vi "VHistory - History Info.vi"(7 "VC Handle":T2=-1, 8 "error in":errorcluster, 11 "name_spec":string) -> (0 "error out":errorcluster, 1 "valid history":bool, 2 "history info":T1 {"oldest timestamp" format="%<%H:%M:%S%2u\n%d/%m/%Y>T"; "NewVals mode"."last read time" format="%<%H:%M:%S%2u\n%d/%m/%Y>T"; "newest timestamp" format="%<%H:%M:%S%2u\n%d/%m/%Y>T"}, 3 "dup name_spec":string, 4 "more data":cluster{"store Writer IDs":bool})   [LabVIEW 2021]
doc: "This VI returns information about a variable history. The VI does not return an error if the specified variable does not have a history attached. Refer to the VI help for more details.\n\n<b>VC Handle</b> specifies the handle of the variable context. To operate on a global variable, pass -1 to this input. This input is ignored if the <b>name_spec</b> control refers to a variable by an alias.\n\n<b>name_spec</b> is the name specifier of the desired variable. Usually, it is merely a variable name; however, its generic format is '[name][=alias]', where either 'name' or '=alias' can be omitted but not both.\n\n<b>history info</b> indicator returns information about both the configuration and state of the history.\n\n<b>valid history</b> indicator returns TRUE if the variable has a history attached.\n\n<b>more data</b> indicator is a cluster containing only the <b>store Writer IDs</b> member, which indicates whether the history stores writer IDs.\n\n::: CalcExpress Toolkit :::\nCopyright (c) 2000-2026 Konstantin Shifershteyn. All rights reserved."
uses:
  cetypes.llb/VarMan Variable Context Handle.ctl
  cetypes.llb/VarMan History Info.ctl
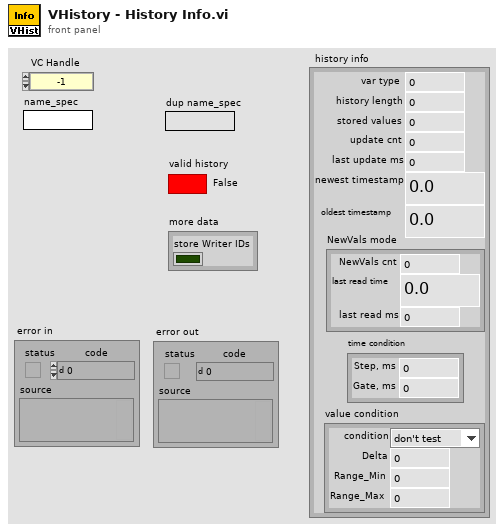
[diagram p1: front panel]
types:
  T1 = typedef "VarMan History Info.ctl" = cluster{"var type":u32, "history length":u32, "stored values":u32, "update cnt":u32, "last update ms":u32, "newest timestamp":dbl, "oldest timestamp":dbl, "NewVals mode":cluster{"NewVals cnt":u32, "last read time":dbl, "last read ms":u32}, "time condition":cluster{"Step, ms":u32, "Gate, ms":u32}, "value condition":cluster{"condition":enum32{"don't test", "changed", "abs deviation", "rel deviation", "out of range", "within range"}, "Delta":dbl, "Range_Min":dbl, "Range_Max":dbl}}
  T2 = typedef "VarMan Variable Context Handle.ctl" = i32
  T3 = enum32{"nop", "create", "destroy", "reset", "get info", "config", "create_wrid"}
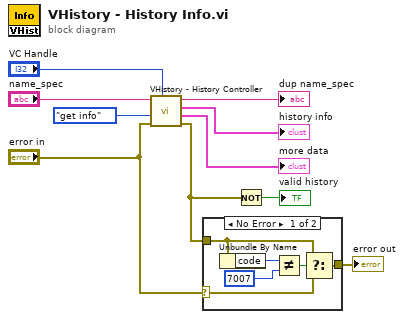
[diagram p0: block diagram]
diagram:
  n1 = call "VHistory - History Controller.vi"("VC Handle"="VC Handle", "error in"="error in", "cmd (nop:default)"=T3."get info", "name_spec"="name_spec") -> ("error out"=w3:errorcluster, "more data"=→"more data":cluster{"store Writer IDs":bool}, "history info"=→"history info":T1, "dup name_spec"=→"dup name_spec":string)  [unwired: 4 in]
  n2 = case shown="No Error" "error in" {
    selector: "error in" -> [w11 w17]
    tunnel: w3 -> [w13 _]
    tunnel: [w12 w17] -> w5
    frame No Error {
      n3 = Unbundle By Name(w13) -> ("code"=w16:i32)
      n4 = Not Equal?(x=w16, y=7007) -> (x != y?=w14:bool)
      n5 = Select(t=w13, s=w14, f=w11) -> (s? t:f=w12:errorcluster)
    }
    frame Error {
    }
  }
  "error out" <- w5
  n6 = Not(x=w3) -> (.not. x?=→"valid history":bool)
